vi "EllipRegionConstraint_New.vi"(6 "Constraint Data Cluster":variant, 8 "Rotation":T1={"VALUE"=0.0, "COS"=1.0, "SIN"=0.0} {"SIN" format="%13.4f"; "COS" format="%13.4f"; "VALUE" format="%13.4f"}, 9 "Y Width":dbl, 10 "X Width":dbl, 11 "Center":T2 {"Y" format="%14.3f"; "X" format="%14.3f"}) -> (3 "ELLIP_REGION_CONSTRAINT":T3={"Center"={"X"=0.0, "Y"=0.0}, "Radii"={"X"=0.0, "Y"=0.0}, "Constraint"=variant, "Constraint Type"=enum."DIFF DRIVE KINEMATICS", "IM UNIQUE"=FALSE} {"Radii"."Y" format="%14.3f"; "Radii"."X" format="%14.3f"; "Center"."Y" format="%14.3f"; "Center"."X" format="%14.3f"})   [LabVIEW 2019, in "Trajectory_Library.lvlib"]
doc: "Constructs a new EllipticalRegionConstraint.\n\nParameters:\n - center -- The center of the ellipse in which to enforce the constraint.\n - xWidth -- The width of the ellipse in which to enforce the constraint.\n - yWidth -- The height of the ellipse in which to enforce the constraint.\n - rotation -- The rotation to apply to all radii around the origin.\n - constraint -- The constraint to enforce when the robot is within the region.\n\nReturns\n - Ellip Region Constraint - Constraint data structure."
uses:
  Trajectory_Library.lvlib
  TypeDef/TRANSLATION2D.ctl
  Enum/TRAJ_CONSTRAINT_TYPES_ENUM.ctl
  TypeDef/TRAJ_CONSTRAINT_ELLIP_REGION.ctl
  TypeDef/ROTATION2D.ctl
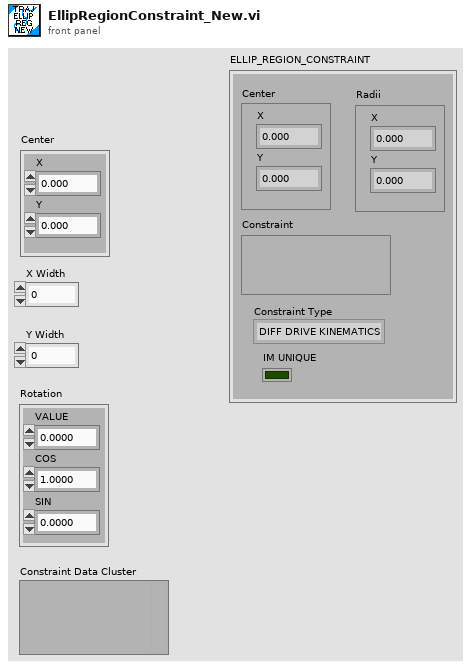
[diagram p1: front panel]
types:
  T1 = typedef "Trajectory_Library.lvlib/ROTATION2D.ctl" = cluster{"VALUE":dbl, "COS":dbl, "SIN":dbl}
  T2 = typedef "Trajectory_Library.lvlib/TRANSLATION2D.ctl" = cluster{"X":dbl, "Y":dbl}
  T3 = typedef "Trajectory_Library.lvlib/TRAJ_CONSTRAINT_ELLIP_REGION.ctl" = cluster{"Center":T2, "Radii":T2, "Constraint":variant, "Constraint Type":T4, "IM UNIQUE":bool}
  T4 = typedef "Trajectory_Library.lvlib/TRAJ_CONSTRAINT_TYPES_ENUM.ctl" = enum16{"UNDEFINED", "DIFF DRIVE KINEMATICS", "DIFF DRIVE VOLTAGE", "CENTRIPITAL ACCEL", "MECA DRIVE KINEMATICS", "SWERVE DRIVE KINEMATICS", "MAXIMUM VELOCITY", "ELLIPTICAL REGION", "RECTANGULAR REGION"}
  T5 = typedef "WPILib_Math.lvlib/TRANSLATION2D.ctl" = cluster{"X":dbl, "Y":dbl}
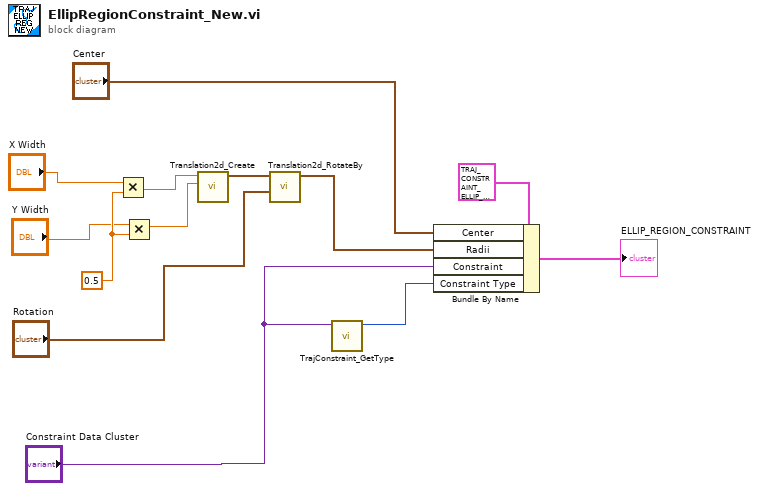
[diagram p0: block diagram]
diagram:
  w9 = 0.5 ("y")
  n1 = Multiply(x="X Width", y=w9) -> (x*y=w6:dbl)
  n2 = Multiply(x="Y Width", y=w9) -> (x*y=w5:dbl)
  n3 = call "Translation2d_Create.vi"("Y"=w5, "X"=w6) -> ("TRANSLATION"=w4:T5)  [unwired: 9 in]
  n4 = call "Translation2d_RotateBy.vi"("other Rotation"="Rotation", "In Translation"=w4) -> ("Out Translation"=w2:T2)  [unwired: 9 in]
  n5 = call "TrajConstraint_GetType.vi"("Trajectory Constraint"="Constraint Data Cluster") -> ("Trajectory Constraint Type"=w10:T4)  [unwired: 9 in, 1 out]
  n6 = Bundle By Name(cluster=T3 {"Center"={"X"=0.0, "Y"=0.0}, "Radii"={"X"=0.0, "Y"=0.0}, "Constraint"=variant, "Constraint Type"=enum."DIFF DRIVE KINEMATICS", "IM UNIQUE"=FALSE} ("ELLIP_REGION_CONSTRAINT"), "Center"="Center", "Radii"=w2, "Constraint"="Constraint Data Cluster", "Constraint Type"=w10) -> (→"ELLIP_REGION_CONSTRAINT":T3)
